vi "Fix Item IDs.vi"(7 "Reload Source?":bool, 8 "error in (no error)":errorcluster, 9 "Saved Item Data":refnum<class "Item.lvclass">[](array[class]), 11 "New Item Data":refnum<class "Item.lvclass">[](array[class])) -> (0 "error out":errorcluster, 1 "Saved Item Data out":refnum<class "Item.lvclass">[](array[class]), 3 "New Item Data out":refnum<class "Item.lvclass">[](array[class]))   [LabVIEW 2020, in "VI Properties Editor.lvlib"]
doc: "Fixes the Item IDs of items in the case of a source being reloaded."
uses:
  VI Properties Editor.lvlib
  Classes/Item/Item.lvclass
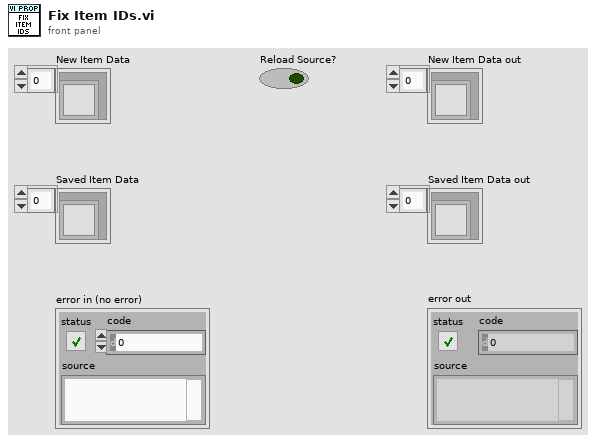
[diagram p1: front panel]
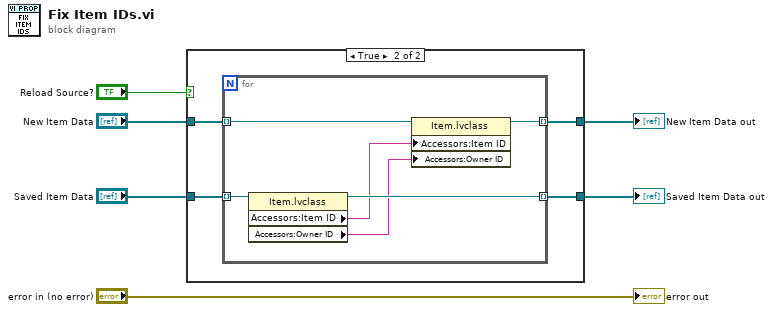
[diagram p0: block diagram]
diagram:
  n1 = case shown="True" "Reload Source?" {
    tunnel: "New Item Data" -> [_ w11]
    tunnel: [w7 w10] -> w5
    tunnel: "Saved Item Data" -> [w7 w9]
    tunnel: [w7 w8] -> w3
    frame False {
    }
    frame True {
      n2 = for {
        tunnel: w11 -> [w16] mode=indexing
        tunnel: [w14] -> w10 mode=indexing
        tunnel: w9 -> [w15] mode=indexing
        tunnel: [w17] -> w8 mode=indexing
        n3 = property class="Item.lvclass"(reference=w15) -> (reference out=w17:refnum<class "Item.lvclass">, "Accessors:Item ID"=w13:string, "Accessors:Owner ID"=w12:string)  [unwired: 1 in, 1 out]
        n4 = property class="Item.lvclass"(reference=w16, "Accessors:Item ID"=w13, "Accessors:Owner ID"=w12) -> (reference out=w14:refnum<class "Item.lvclass">)  [unwired: 1 in, 1 out]
      }
    }
  }
  "New Item Data out" <- w5
  "Saved Item Data out" <- w3
  "error out" <- "error in (no error)"
